vi "Simple navdata with gotoxy.vi"() -> ()   [LabVIEW 2014]
doc: "Very simple example showing how to use the base VIs to control the AR Drone and receive and display navigation data."
uses:
  <vilib>/LVH/AR Drone Toolkit/Decode NavData/Typedefs/NavData Demo.ctl
  <vilib>/LVH/AR Drone Toolkit/AR Drone.lvlib
  <vilib>/ptbypt/NI_PtbyPt.lvlib
panel:
  out "error out":errorcluster
  in  "device ID":i32=3
  in  "manual":bool
  out "Control Cluster 2":T1
  out "XY Graph":cluster{"Y":dbl[], "Y":dbl[]}[](graph)
  in  "stop 2":bool
  in  "Emergency Landing 2":bool
  in  "Take Off/Land 2":bool
  in  "Hover 2":bool
  in  "Y goal":dbl
  in  "X goal":dbl
  out "Battery Remaining":dbl(slide) scale=0.0..100.0
  out "NavData Out":T2
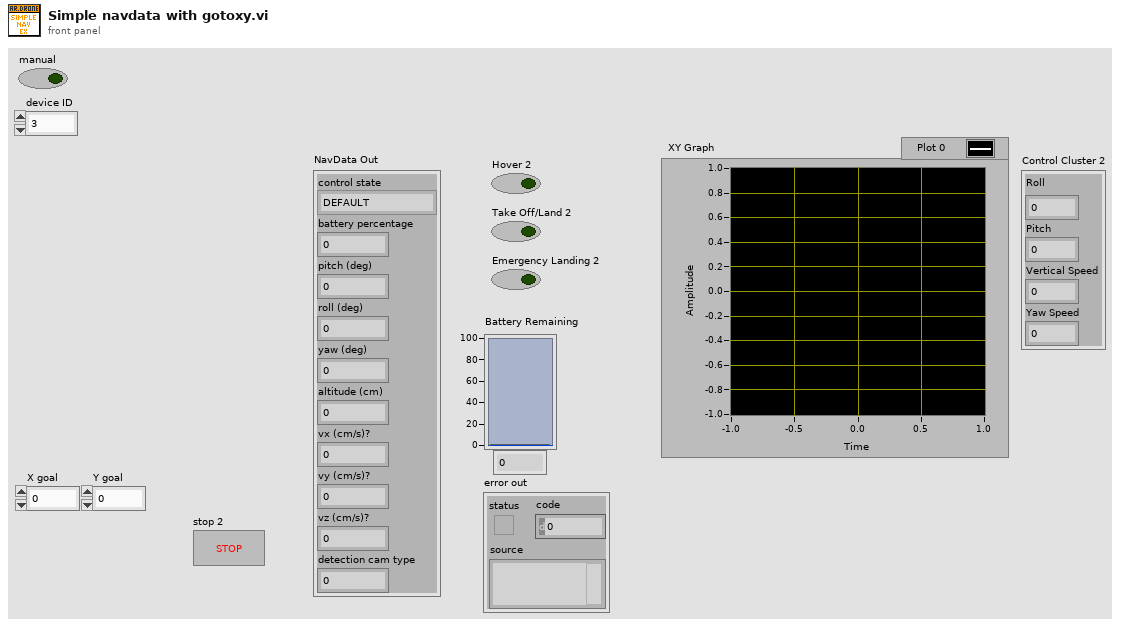
[diagram p1: front panel]
types:
  T1 = cluster{"Roll":sgl, "Pitch":sgl, "Vertical Speed":sgl, "Yaw Speed":sgl}
  T2 = typedef "AR Drone.lvlib/NavData Demo.ctl" = cluster{"control state":enum32{"DEFAULT", "INIT", "LANDING", "FLYING", "HOVERING", "TEST", "TRANS_TAKEOFF", "TRANS_GOTOFIX", "TRANS_LANDING"}, "battery percentage":u32, "pitch (deg)":sgl, "roll (deg)":sgl, "yaw (deg)":sgl, "altitude (cm)":u32, "vx (cm/s)?":sgl, "vy (cm/s)?":sgl, "vz (cm/s)?":sgl, "detection cam type":u32}
  T3 = typedef "AR Drone.lvlib/AR Drone Resource.ctl" = cluster{"UDP Control Connection":refnum<k16>, "UDP NavData Connection":refnum<k16>, "UDP Video Connection (Drone 1.0)":refnum<k16>, "TCP Video Connection (Drone 2.0)":refnum<k5>, "TCP Control Port Connection":refnum<k5>, "Drone IP address":string, "Drone Command Port":u16, "Drone NavData Port":u16, "Drone Vid Stream Port":u16, "Drone TCP Control Port":u16, "Home IP address":string, "Home Command Port":u16, "Home NavData Port":u16, "Home Vid Stream Port":u16, "Drone Version":i32, "Drone Index":i32, "Command Sequence":i32}
  T4 = cluster{"Roll":dbl, "Pitch":dbl, "Vertical Speed":dbl, "Yaw Speed":dbl}
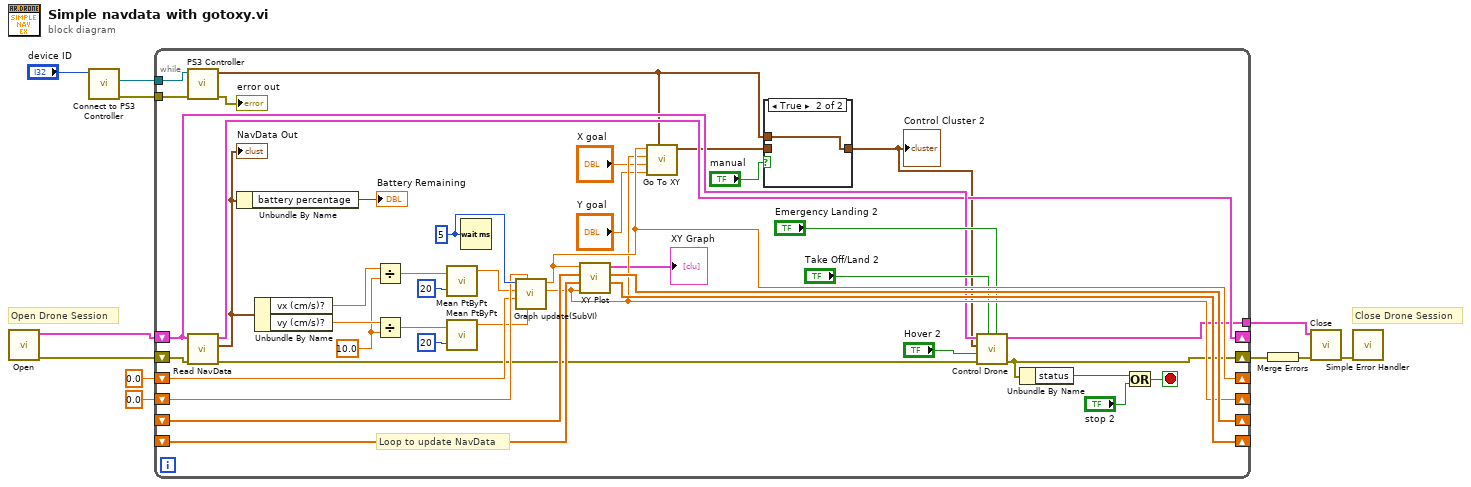
[diagram p0: block diagram]
diagram:
  # "Close Drone Session"
  # "Open Drone Session"
  n1 = call <vilib>:"Open.vi"() -> ("error out"=w10:errorcluster, "AR Drone Resource"=w11:T3)  [unwired: 10 in]
  n2 = call "Connect to PS3 Controller.vi"("device ID"="device ID") -> ("error out"=w3:errorcluster, "device ID 2"=w2:refnum<k1>)  [unwired: 7 in, 1 out]
  n3 = while {
    shift-right: [w32] -> _
    shift-left: w11 -> [w35]
    shift-right: [w12] -> w5
    shift-left: w10 -> [w34]
    shift-right: [w50] -> _
    shift-left: _ -> [w47]
    shift-right: [w49] -> _
    shift-left: _ -> [w48]
    shift-right: [w44] -> _
    shift-left: 0.0 ("Numeric 3") -> [w45]
    shift-right: [w43] -> _
    shift-left: 0.0 ("Numeric out") -> [w46]
    tunnel: [w30] -> w4
    tunnel: w3 -> [w18]
    tunnel: w2 -> [w17]
    stop <- w33 stop-if-true
    w23 = sgl 10.0 ("y")
    w52 = u32 5 ("milliseconds to wait")
    # "Loop to update NavData"
    n4 = call "PS3 Controller.vi"("error in (no error)"=w18, "device ID"=w17) -> ("error out"=→"error out":errorcluster, "Control cluster"=w14:T4)  [unwired: 6 in, 2 out]
    n5 = call <vilib>:"Read NavData.vi"("error in (no error)"=w34, "AR Drone Resource"=w35) -> ("error out"=w13:errorcluster, "NavData Out"=w51:T2, "AR Drone Resource Out"=w32:T3)  [unwired: 7 in]
    "NavData Out" <- w51
    n6 = Unbundle By Name(w51) -> ("battery percentage"=→"Battery Remaining":u32)
    n7 = Unbundle By Name(w51) -> ("vx (cm/s)?"=w25:sgl, "vy (cm/s)?"=w24:sgl)
    n8 = Divide(x=w25, y=w23) -> (x/y=w21:sgl)
    n9 = Divide(x=w24, y=w23) -> (x/y=w22:sgl)
    n10 = call <vilib>:"Mean PtByPt.vi"("x"=w21, "sample length"=20) -> ("mean"=w28:dbl)  [unwired: 2 in, 1 out]
    n11 = call <vilib>:"Mean PtByPt.vi"("x"=w22, "sample length"=20) -> ("mean"=w26:dbl)  [unwired: 2 in, 1 out]
    n12 = Wait (ms)(milliseconds to wait=w52) -> ()  [unwired: 1 out]
    n13 = call "Graph update(SubVI).vi"("vy (cm/s)?"=w26, "Numeric 4"=w46, "Numeric in"=w45, "vx (cm/s)?"=w28, "milliseconds to wait"=w52) -> ("Numeric out"=w43:dbl, "Numeric 3"=w44:dbl)  [unwired: 5 in]
    n14 = call "XY Plot.vi"("X"=w44, "X array"=w47, "Y array"=w48, "Y"=w43) -> ("XY Graph"=→"XY Graph":cluster{"Y":dbl[], "Y":dbl[]}[], "X array"=w50:dbl[], "Y array"=w49:dbl[])  [unwired: 2 in, 1 out]
    n15 = call "Go To XY.vi"("Control Cluster"=w14, "Y goal"="Y goal", "X goal"="X goal", "Y current"=w43, "X current"=w44) -> ("Control Cluster"=w20:T1)  [unwired: 6 in]
    n16 = case shown="True" "manual" {
      tunnel: [w54 w55] -> w15
      tunnel: w20 -> [w54 _]
      tunnel: w14 -> [_ w55]
      frame False {
      }
      frame True {
      }
    }
    "Control Cluster 2" <- w15
    n17 = call <vilib>:"Control Drone.vi"("Emergency Landing"="Emergency Landing 2", "Takeoff/Land"="Take Off/Land 2", "error in (no error)"=w13, "Hover"="Hover 2", "Control Cluster"=w15, "AR Drone Resource"=w35) -> ("error out"=w12:errorcluster, "AR Drone Resource Out"=w30:T3)  [unwired: 4 in]
    n18 = Unbundle By Name(w12) -> ("status"=w37:bool)
    n19 = Or(x=w37, y="stop 2") -> (x .or. y?=w33:bool)
  }
  n20 = Merge Errors(w5) -> (w9:errorcluster)
  n21 = call <vilib>:"Close.vi"("error in (no error)"=w9, "AR Drone Resource"=w4) -> ("error out"=w8:errorcluster)  [unwired: 9 in]
  n22 = call <vilib>:"Simple Error Handler.vi"("error in (no error)"=w8) -> ()  [unwired: 4 in, 5 out]
